vi "Extract Single File.vi"(5 "Overwrite":bool, 7 "Return as String (F: Extract to File)":bool, 8 "error in (no error)":errorcluster, 9 "name or relative path (\"\": use output file name)":string, 10 "File output Path (extract to temp file)":path, 11 "Zip File Path":path) -> (0 "error out":errorcluster, 1 "String":string, 2 "Extracted File Path":path, 3 "dup Zip File Path":path)   [LabVIEW 2020, in "Command-Line Zip.lvlib"]
uses:
  Command-Line Zip.lvlib
  <userlib>/_OpenG.lib/file/file.llb/Valid Path - Traditional__ogtk.vi
  <userlib>/_OpenG.lib/file/file.llb/openg_file.lvlib
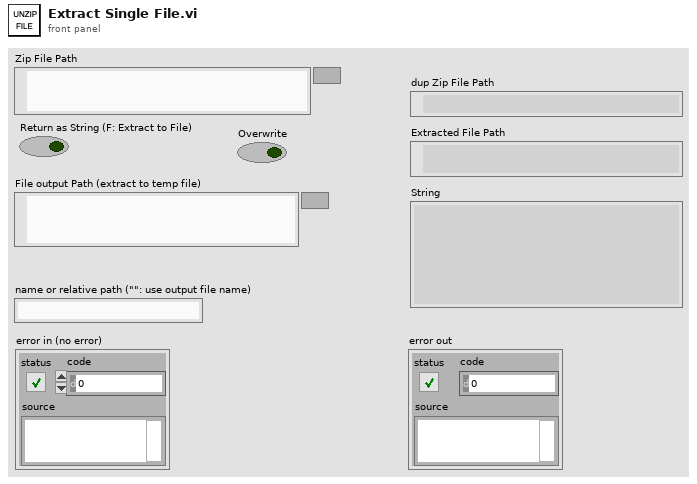
[diagram p1: front panel]
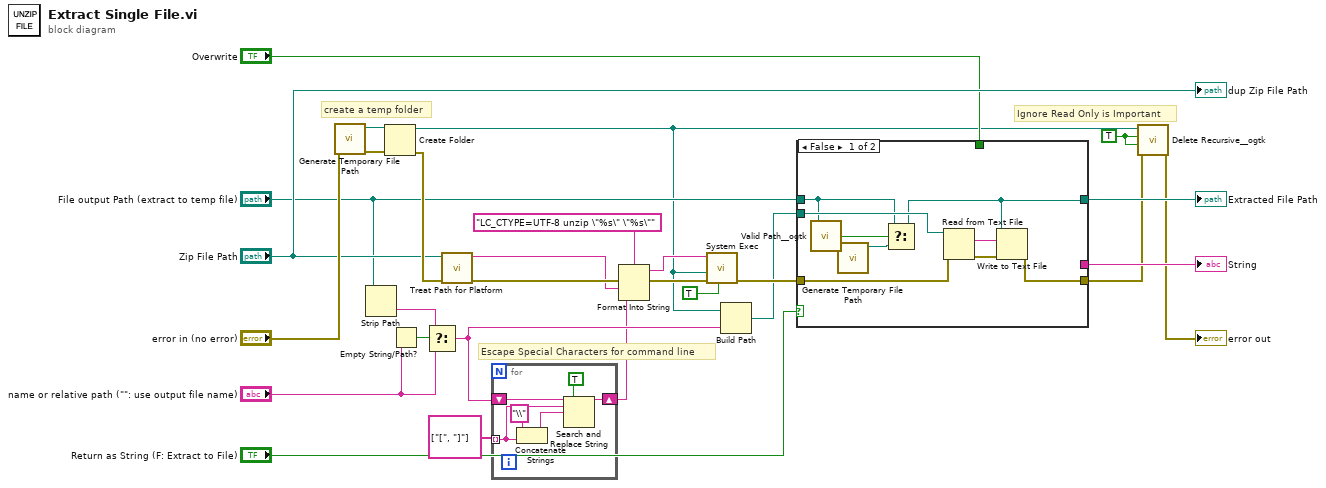
[diagram p0: block diagram]
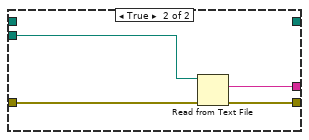
[diagram p2: hidden frame]
diagram:
  w7 = TRUE ("Recursive? (FALSE)")
  # "Ignore Read Only is Important"
  # "Escape Special Characters for command line"
  # "create a temp folder"
  n1 = call <vilib>:"Generate Temporary File Path.vi"("error in (no error)"="error in (no error)") -> ("error out"=w20:errorcluster, "Unique Temporary File Path"=w21:path)  [unwired: 9 in]
  n2 = Strip Path(path="File output Path (extract to temp file)") -> (name=w10:string)  [unwired: 1 out]
  n3 = Create Folder(path (use dialog)=w21, error in=w20) -> (created path=w4:path, error out=w22:errorcluster)  [unwired: 1 in, 1 out]
  n4 = Empty String/Path?(string/path="name or relative path (\"\": use output file name)") -> (empty?=w11:bool)
  n5 = Select(t=w10, s=w11, f="name or relative path (\"\": use output file name)") -> (s? t:f=w2:string)
  n6 = call "Treat Path for Platform.vi"("error in (no error)"=w22, "File Path"="Zip File Path") -> ("error out"=w19:errorcluster, "Path for CLI"=w18:string)  [unwired: 8 in]
  n7 = for {
    shift-right: [w32] -> w1
    shift-left: w2 -> [w34]
    tunnel: string[] ["[", "]"] -> [w30] mode=indexing
    n8 = Concatenate Strings("\\" ("string"), w30) -> (w29:string)
    n9 = Search and Replace String(replace all?=TRUE ("replace all? (F)"), input string=w34, search string=w30, replace string=w29) -> (result string=w32:string)  [unwired: 4 in, 3 out]
  }
  n10 = Format Into String(format string="LC_CTYPE=UTF-8 unzip \"%s\" \"%s\"" ("command line"), error in=w19, w18, w1) -> (resulting string=w15:string, error out=w16:errorcluster)  [unwired: 1 in]
  n11 = call <vilib>:"System Exec.vi"("run minimized? (F)"=TRUE, "error in (no error)"=w16, "working directory"=w4, "command line"=w15) -> ("error out"=w24:errorcluster)  [unwired: 4 in, 3 out]
  n12 = Build Path(base path=w4, name or relative path=w2) -> (appended path=w23:path)
  n13 = case shown="False" "Return as String (F: Extract to File)" {
    tunnel: w23 -> [w38 w46]
    tunnel: "File output Path (extract to temp file)" -> [w35 _]
    tunnel: w24 -> [w42 w47]
    tunnel: [w43 w45] -> w5
    tunnel: [_ w44] -> w26
    tunnel: [w36 _] -> w28
    tunnel: "Overwrite" -> [_ _]
    frame False {
      n14 = call-poly <userlib>:"Valid Path__ogtk.vi"("path"=w35) -> ("valid"=w39:bool)
      n15 = call <vilib>:"Generate Temporary File Path.vi"() -> ("Unique Temporary File Path"=w37:path)  [unwired: 10 in, 1 out]
      n16 = Select(t=w35, s=w39, f=w37) -> (s? t:f=w36:path)
      n17 = Read from Text File(file (use dialog)=w38, error in=w42) -> (text=w40:string, error out=w41:errorcluster)  [unwired: 2 in, 2 out]
      n18 = Write to Text File(file (use dialog)=w36, text=w40, error in=w41) -> (error out=w43:errorcluster)  [unwired: 1 in, 2 out]
    }
    frame True {
      n19 = Read from Text File(file (use dialog)=w46, error in=w47) -> (text=w44:string, error out=w45:errorcluster)  [unwired: 2 in, 2 out]
    }
  }
  "Extracted File Path" <- w28
  "String" <- w26
  n20 = call <userlib>:"Delete Recursive__ogtk.vi"("error in (no error)"=w5, "Ignore Read-Only? (FALSE)"=w7, "Recursive? (FALSE)"=w7, "Path"=w4) -> ("error out"=→"error out":errorcluster)  [unwired: 6 in, 1 out]
  "dup Zip File Path" <- "Zip File Path"
